vi "Test_Engine.vi"() -> ()   [LabVIEW 2026]
doc: "DAQ_Engine 테스트: Start, Log On, Log Off(이때 최신 데이터 확인), Stop, Exit."
panel:
  out "engine error":errorcluster
  out "error out":errorcluster
  out "Mid Message":string
  out "Final Message":string
  out "Log File":path
  out "Logging":bool
  out "Running":bool
  out "dt":dbl
  out "Rows":i32
  out "Values":dbl[](array[numeric])
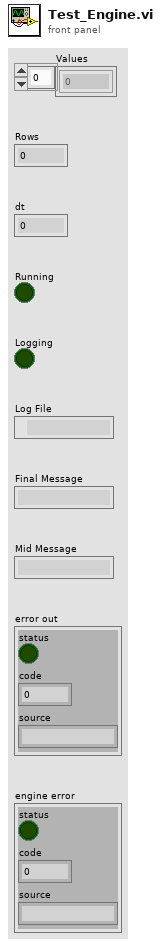
[diagram p1: front panel]
types:
  T1 = enum16{"Start", "Stop", "Config", "Log On", "Log Off", "Exit"}
  T2 = cluster{"Cmd":enum16{"Start", "Stop", "Config", "Log On", "Log Off", "Exit"}, "Settings":cluster{"Sample Rate (Hz)":dbl, "Samples per Channel":i32, "Chassis 1 Channels":string, "Chassis 2 Channels":string, "Save Folder":path}, "Channels":cluster{"Name":string, "Value":dbl, "High Limit":dbl, "Low Limit":dbl, "Save":bool, "Graph":bool, "Scale Min":dbl, "Scale Max":dbl, "Unit":string}[]}
  T3 = cluster{"Data":dbl[][], "Values":dbl[], "dt":dbl, "Running":bool, "Logging":bool, "Message":string, "Log File":path}
  T4 = cluster{"Name":string, "Value":dbl, "High Limit":dbl, "Low Limit":dbl, "Save":bool, "Graph":bool, "Scale Min":dbl, "Scale Max":dbl, "Unit":string}[]
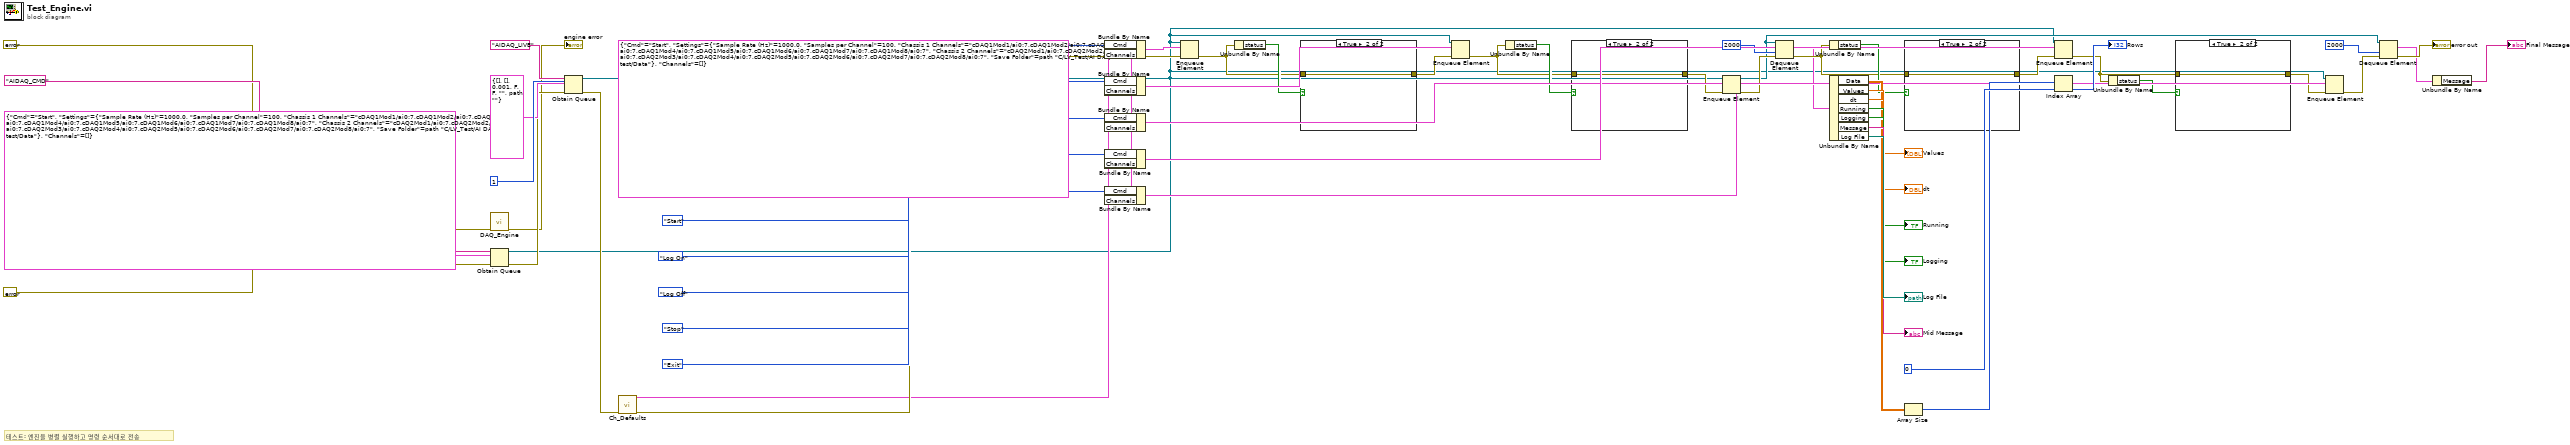
[diagram p0: block diagram]
diagram:
  w15 = T2 {"Cmd"=enum."Start", "Settings"={"Sample Rate (Hz)"=1000.0, "Samples per Channel"=100, "Chassis 1 Channels"="cDAQ1Mod1/ai0:7,cDAQ1Mod2/ai0:7,cDAQ1Mod3/ai0:7,cDAQ1Mod4/ai0:7,cDAQ1Mod5/ai0:7,cDAQ1Mod6/ai0:7,cDAQ1Mod7/ai0:7,cDAQ1Mod8/ai0:7", "Chassis 2 Channels"="cDAQ2Mod1/ai0:7,cDAQ2Mod2/ai0:7,cDAQ2Mod3/ai0:7,cDAQ2Mod4/ai0:7,cDAQ2Mod5/ai0:7,cDAQ2Mod6/ai0:7,cDAQ2Mod7/ai0:7,cDAQ2Mod8/ai0:7", "Save Folder"=path "C:/LV_Test/AI DAQ md test/Data"}, "Channels"=[]}
  # "테스트: 엔진을 병렬 실행하고 명령 순서대로 전송"
  n1 = call "DAQ_Engine.vi"("error in"=errorcluster {"status"=FALSE, "code"=0, "source"=""}) -> ("error out"=→"engine error":errorcluster)  [unwired: 14 in]
  n2 = Obtain Queue(name (unnamed)="AIDAQ_CMD", element data type=T2 {"Cmd"=enum."Start", "Settings"={"Sample Rate (Hz)"=1000.0, "Samples per Channel"=100, "Chassis 1 Channels"="cDAQ1Mod1/ai0:7,cDAQ1Mod2/ai0:7,cDAQ1Mod3/ai0:7,cDAQ1Mod4/ai0:7,cDAQ1Mod5/ai0:7,cDAQ1Mod6/ai0:7,cDAQ1Mod7/ai0:7,cDAQ1Mod8/ai0:7", "Chassis 2 Channels"="cDAQ2Mod1/ai0:7,cDAQ2Mod2/ai0:7,cDAQ2Mod3/ai0:7,cDAQ2Mod4/ai0:7,cDAQ2Mod5/ai0:7,cDAQ2Mod6/ai0:7,cDAQ2Mod7/ai0:7,cDAQ2Mod8/ai0:7", "Save Folder"=path "C:/LV_Test/AI DAQ md test/Data"}, "Channels"=[]}, error in (no error)=errorcluster {"status"=FALSE, "code"=0, "source"=""}) -> (queue out=w6:refnum<queue>, error out=w7:errorcluster)  [unwired: 2 in, 1 out]
  n3 = Obtain Queue(max queue size (-1, unlimited)=1, name (unnamed)="AIDAQ_LIVE", element data type=T3 {"Data"=[], "Values"=[], "dt"=0.001, "Running"=FALSE, "Logging"=FALSE, "Message"="", "Log File"=path ""}, error in (no error)=w7) -> (queue out=w11:refnum<queue>, error out=w12:errorcluster)  [unwired: 1 in, 1 out]
  n4 = call "Ch_Defaults.vi"("error in"=w12) -> ("Channels"=w13:T4, "error out"=w14:errorcluster)  [unwired: 13 in]
  n5 = Bundle By Name(cluster=w15, "Cmd"=T1."Start", "Channels"=w13) -> (w17:T2)
  n6 = Bundle By Name(cluster=w15, "Cmd"=T1."Log On", "Channels"=w13) -> (w22:T2)
  n7 = Bundle By Name(cluster=w15, "Cmd"=T1."Log Off", "Channels"=w13) -> (w27:T2)
  n8 = Bundle By Name(cluster=w15, "Cmd"=T1."Stop", "Channels"=w13) -> (w35:T2)
  n9 = Bundle By Name(cluster=w15, "Cmd"=T1."Exit", "Channels"=w13) -> (w40:T2)
  n10 = Enqueue Element(queue=w6, element=w17, error in (no error)=w14) -> (error out=w18:errorcluster)  [unwired: 1 in, 2 out]
  n11 = Unbundle By Name(w18) -> ("status"=w19:bool)
  n12 = case shown="True" w19 {
    tunnel: w18 -> [w56 w58]
    tunnel: [w56 w58] -> w20
    frame False {
      # "대기"
      n13 = Wait (ms)(milliseconds to wait=1500) -> ()  [unwired: 1 out]
    }
    frame True {
    }
  }
  n14 = Enqueue Element(queue=w6, element=w22, error in (no error)=w20) -> (error out=w23:errorcluster)  [unwired: 1 in, 2 out]
  n15 = Unbundle By Name(w23) -> ("status"=w24:bool)
  n16 = case shown="True" w24 {
    tunnel: w23 -> [w59 w61]
    tunnel: [w59 w61] -> w25
    frame False {
      # "대기"
      n17 = Wait (ms)(milliseconds to wait=1000) -> ()  [unwired: 1 out]
    }
    frame True {
    }
  }
  n18 = Enqueue Element(queue=w6, element=w27, error in (no error)=w25) -> (error out=w28:errorcluster)  [unwired: 1 in, 2 out]
  n19 = Dequeue Element(queue=w11, timeout in ms (-1)=2000, error in (no error)=w28) -> (element=w30:T3, error out=w31:errorcluster)  [unwired: 2 out]
  n20 = Unbundle By Name(w31) -> ("status"=w32:bool)
  n21 = Unbundle By Name(w30) -> ("Data"=w45:dbl[][], "Values"=→"Values":dbl[], "dt"=→"dt":dbl, "Running"=→"Running":bool, "Logging"=→"Logging":bool, "Message"=→"Mid Message":string, "Log File"=→"Log File":path)
  n22 = case shown="True" w32 {
    tunnel: w31 -> [w62 w64]
    tunnel: [w62 w64] -> w33
    frame False {
      # "대기"
      n23 = Wait (ms)(milliseconds to wait=300) -> ()  [unwired: 1 out]
    }
    frame True {
    }
  }
  n24 = Array Size(array=w45) -> (size(s)=w52:i32[])
  n25 = Enqueue Element(queue=w6, element=w35, error in (no error)=w33) -> (error out=w36:errorcluster)  [unwired: 1 in, 2 out]
  n26 = Index Array(array=w52, index=0) -> (element=→"Rows":i32)
  n27 = Unbundle By Name(w36) -> ("status"=w37:bool)
  n28 = case shown="True" w37 {
    tunnel: w36 -> [w65 w67]
    tunnel: [w65 w67] -> w38
    frame False {
      # "대기"
      n29 = Wait (ms)(milliseconds to wait=800) -> ()  [unwired: 1 out]
    }
    frame True {
    }
  }
  n30 = Enqueue Element(queue=w6, element=w40, error in (no error)=w38) -> (error out=w41:errorcluster)  [unwired: 1 in, 2 out]
  n31 = Dequeue Element(queue=w11, timeout in ms (-1)=2000, error in (no error)=w41) -> (element=w43:T3, error out=→"error out":errorcluster)  [unwired: 2 out]
  n32 = Unbundle By Name(w43) -> ("Message"=→"Final Message":string)
